vi "Time Profile Graph formation.vi"(8 "time":dbl[](array[numeric]), 11 "CP Probability":dbl[][](array[numeric])) -> (3 "Time Profile Graph":cluster{"time":dbl[], dbl[]}[](graph))   [LabVIEW 2018]
panel:
  out "配列":cluster{i32[], dbl[]}[](array[cluster])
  out "サイズ":i32[](array[numeric])
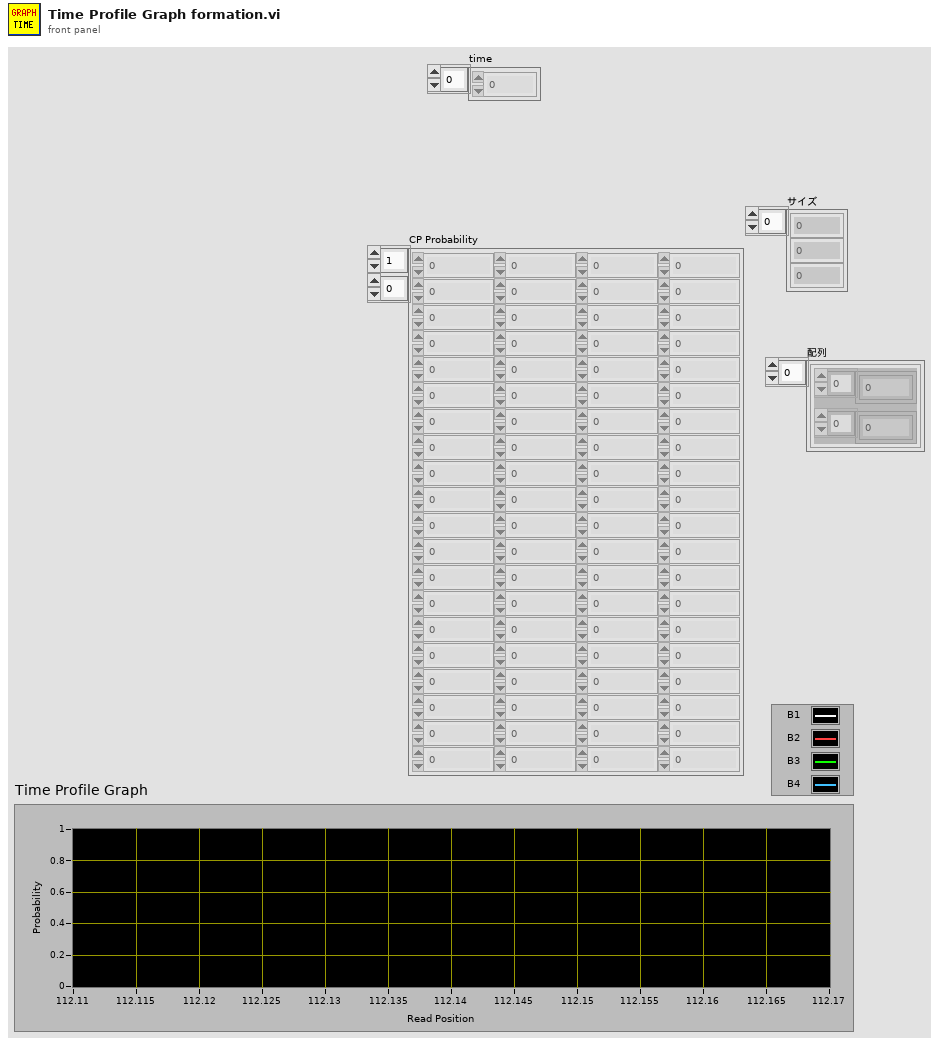
[diagram p1: front panel]
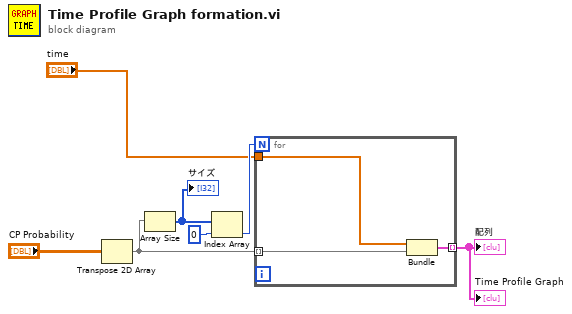
[diagram p0: block diagram]
diagram:
  n1 = Transpose 2D Array(2D array="CP Probability") -> (transposed array=w4:dbl[][])
  n2 = Array Size(array=w4) -> (size(s)=w6:i32[])
  "サイズ" <- w6
  n3 = Index Array(array=w6, index=0 ("指標")) -> (element=w3:i32)
  n4 = for {
    N: w3 -> [_]
    tunnel: w4 -> [w10] mode=indexing
    tunnel: [w9] -> w2 mode=indexing
    tunnel: "time" -> [w8]
    n5 = Bundle("time"=w8, w10) -> (w9:cluster{"time":dbl[], dbl[]})  [unwired: 1 in]
  }
  "配列" <- w2
  "Time Profile Graph" <- w2
